vi "Lire fichiers config acqui.vi"(2 "error in (no error)":errorcluster caption="entrée d'erreur (pas d'erreur)") -> (0 "error out":errorcluster caption="sortie d'erreur")   [LabVIEW 2022 SP3]
uses:
  Variables globales/Variable glob Leybold.vi
  Variables globales/Variable glob Edwards.vi
  Variables globales/Variable glob Keller.vi
  Variables globales/Variables glob EUROTHERM.vi
  Variables globales/Variable globale compteurs.vi
  <vilib>/Utility/config.llb/NI_LVConfig.lvlib
panel:
  out "chemin complet":path
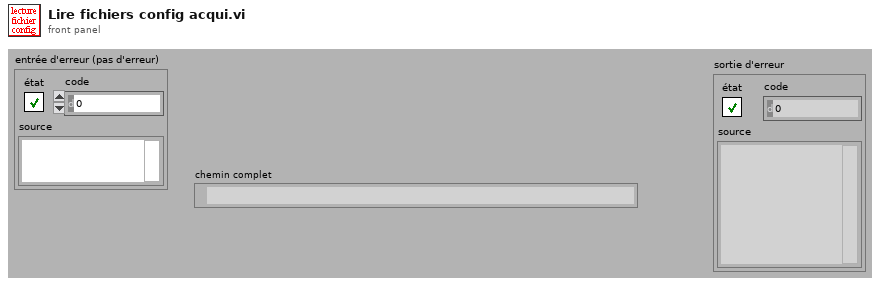
[diagram p1: front panel]
types:
  T1 = typedef "NI_LVConfig.lvlib/Config Data RefNum.ctl" = refnum<k1>
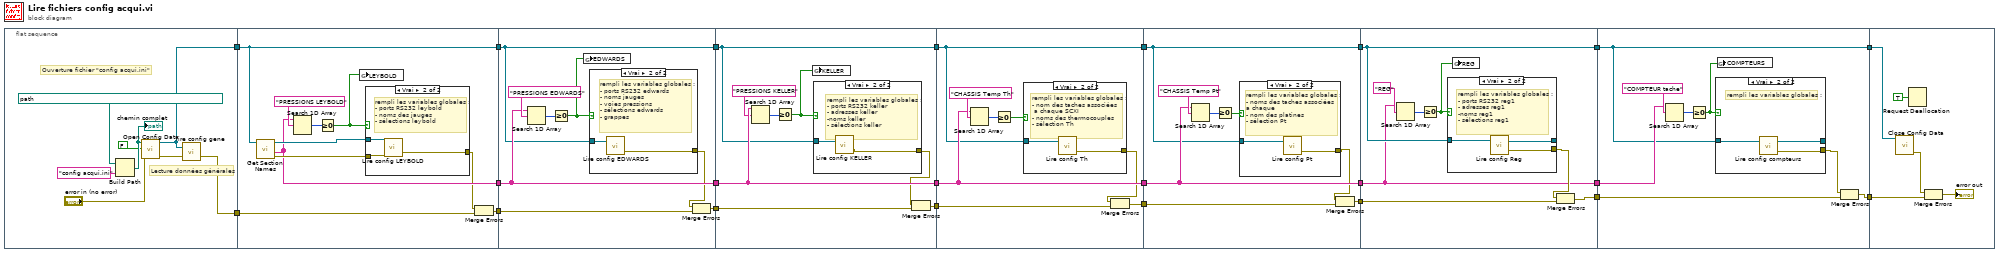
[diagram p0: block diagram]
diagram:
  n1 = flat-sequence {
    tunnel: [w26] -> w17
    tunnel: [w23] -> w16
    tunnel: w17 -> [w33]
    tunnel: [w35] -> w22
    tunnel: w16 -> [w34]
    tunnel: [w34] -> w15
    tunnel: [w31] -> w10
    tunnel: w22 -> [w49]
    tunnel: [w49] -> w21
    tunnel: w15 -> [w48]
    tunnel: [w48] -> w14
    tunnel: w10 -> [w47]
    tunnel: [w45] -> w9
    tunnel: w21 -> [w61]
    tunnel: [w61] -> w20
    tunnel: w14 -> [w58]
    tunnel: [w58] -> w13
    tunnel: w9 -> [w57]
    tunnel: [w55] -> w8
    tunnel: w20 -> [w69]
    tunnel: [w69] -> w19
    tunnel: w13 -> [w68]
    tunnel: [w68] -> w12
    tunnel: w8 -> [w67]
    tunnel: [w65] -> w7
    tunnel: w19 -> [w79]
    tunnel: [w79] -> w18
    tunnel: w12 -> [w78]
    tunnel: [w78] -> w11
    tunnel: w7 -> [w77]
    tunnel: [w75] -> w6
    tunnel: w18 -> [w85]
    tunnel: w11 -> [w89]
    tunnel: [w89] -> w5
    tunnel: w6 -> [w88]
    tunnel: [w87] -> w3
    tunnel: [w85] -> w1
    tunnel: w5 -> [w100]
    tunnel: [w100] -> w4
    tunnel: w3 -> [w98]
    tunnel: [w97] -> w2
    tunnel: w1 -> [w101]
    tunnel: w4 -> [w112]
    tunnel: w2 -> [w111]
    frame #0 {
      # "Lecture données générales"
      # "Ouverture fichier \"config acqui.ini\""
      n2 = Build Path(base path=path "C:/LABVIEW/PRES+TEMP+REG dernière version/Configurations", name or relative path="config acqui.ini" ("nom ou chemin relatif")) -> (appended path=w30:path)
      "chemin complet" <- w30
      n3 = call <vilib>:"Open Config Data.vi"("error in (no error)"="error in (no error)", "create file if necessary (T)"=FALSE ("create file if necessary? (T)"), "configuration file path"=w30) -> ("error out"=w27:errorcluster, "refnum"=w23:T1)  [unwired: 6 in, 1 out]
      n4 = call "lire config gene.vi"("error in"=w27, "refnum"=w23) -> ("error out"=w26:errorcluster)  [unwired: 1 out]
    }
    frame #1 {
      n5 = call <vilib>:"Get Section Names.vi"("refnum"=w34) -> ("error out"=w37:errorcluster, "section names"=w35:string[], "refnum out"=w38:T1)  [unwired: 8 in]
      n6 = Search 1D Array(1D array=w35, element="PRESSIONS LEYBOLD") -> (index of element=w39:i32)  [unwired: 1 in]
      n7 = Greater Or Equal To 0?(x=w39) -> (x >= 0?=w36:bool)
      n8 = global write "Variable glob Leybold.vi" "LEYBOLD"(w36) -> ()
      n9 = case shown="Vrai" w36 {
        tunnel: w38 -> [_ w44]
        tunnel: w37 -> [w41 w43]
        tunnel: [w41 w42] -> w32
        frame False {
          # "Pas de jauges\nLEYBOLD"
        }
        frame True {
          # "rempli les variables globales :\n- ports RS232 leybold\n- noms des jauges\n- sélections leybold"
          n10 = call "Lire config LEYBOLD.vi"("error in (no error)"=w43, "refnum"=w44) -> ("error out"=w42:errorcluster)  [unwired: 1 out]
        }
      }
      n11 = Merge Errors(w32, w33) -> (w31:errorcluster)
    }
    frame #2 {
      n12 = Search 1D Array(1D array=w49, element="PRESSIONS EDWARDS") -> (index of element=w51:i32)  [unwired: 1 in]
      n13 = Greater Or Equal To 0?(x=w51) -> (x >= 0?=w52:bool)
      n14 = global write "Variable glob Edwards.vi" "EDWARDS"(w52) -> ()
      n15 = case shown="Vrai" w52 {
        tunnel: w48 -> [_ w54]
        tunnel: [_ w53] -> w46
        frame False {
          # "Pas de jauges\nEDWARDS"
        }
        frame True {
          # "rempli les variables globales :\n- ports RS232 edwards\n- noms jauges\n- voies pressions\n- sélections edwards\n- grappes"
          n16 = call "Lire config EDWARDS.vi"("refnum"=w54) -> ("error out"=w53:errorcluster)  [unwired: 1 in, 1 out]
        }
      }
      n17 = Merge Errors(w46, w47) -> (w45:errorcluster)
    }
    frame #3 {
      n18 = Search 1D Array(1D array=w61, element="PRESSIONS KELLER") -> (index of element=w62:i32)  [unwired: 1 in]
      n19 = Greater Or Equal To 0?(x=w62) -> (x >= 0?=w59:bool)
      n20 = global write "Variable glob Keller.vi" "KELLER"(w59) -> ()
      n21 = case shown="Vrai" w59 {
        tunnel: w58 -> [_ w64]
        tunnel: [_ w63] -> w56
        frame False {
          # "Pas de jauges\nKELLER"
        }
        frame True {
          # "rempli les variables globales :\n- ports RS232 keller\n- adresses keller\n-noms keller\n- sélections keller"
          n22 = call "Lire config KELLER.vi"("refnum"=w64) -> ("error out"=w63:errorcluster)  [unwired: 1 in, 1 out]
        }
      }
      n23 = Merge Errors(w56, w57) -> (w55:errorcluster)
    }
    frame #4 {
      n24 = Search 1D Array(1D array=w69, element="CHASSIS Temp Th") -> (index of element=w72:i32)  [unwired: 1 in]
      n25 = Greater Or Equal To 0?(x=w72) -> (x >= 0?=w70:bool)
      n26 = case shown="Vrai" w70 {
        tunnel: w68 -> [_ w74]
        tunnel: [_ w73] -> w66
        frame False {
        }
        frame True {
          # "rempli les variables globales :\n- nom des taches associées\n a chaque SCXI\n- noms des thermocouples\n- sélection Th"
          n27 = call "Lire config Th.vi"("refnum"=w74) -> ("error out"=w73:errorcluster)  [unwired: 1 in, 1 out]
        }
      }
      n28 = Merge Errors(w66, w67) -> (w65:errorcluster)
    }
    frame #5 {
      n29 = Search 1D Array(1D array=w79, element="CHASSIS Temp Pt" ("section")) -> (index of element=w82:i32)  [unwired: 1 in]
      n30 = Greater Or Equal To 0?(x=w82) -> (x >= 0?=w81:bool)
      n31 = case shown="Vrai" w81 {
        tunnel: w78 -> [_ w84]
        tunnel: [_ w83] -> w76
        frame False {
        }
        frame True {
          # "rempli les variables globales :\n- noms des taches associées \na chaque \n- nom des platines\n- sélection Pt"
          n32 = call "Lire config Pt.vi"("refnum"=w84) -> ("error out"=w83:errorcluster)  [unwired: 1 in, 1 out]
        }
      }
      n33 = Merge Errors(w76, w77) -> (w75:errorcluster)
    }
    frame #6 {
      n34 = Search 1D Array(1D array=w85, element="REG" ("section")) -> (index of element=w91:i32)  [unwired: 1 in]
      n35 = Greater Or Equal To 0?(x=w91) -> (x >= 0?=w90:bool)
      n36 = case shown="Vrai" w90 {
        tunnel: w89 -> [w93 w96]
        tunnel: [_ w95] -> w86
        tunnel: [w93 w94] -> _
        frame False {
        }
        frame True {
          # "rempli les variables globales :\n- ports RS232 reg1\n- adresses reg1\n-noms reg1\n- sélections reg1"
          n37 = call "Lire config Reg.vi"("refnum"=w96) -> ("error out"=w95:errorcluster, "refnum out"=w94:T1)  [unwired: 1 in]
        }
      }
      n38 = global write "Variables glob EUROTHERM.vi" "REG"(w90) -> ()
      n39 = Merge Errors(w86, w88) -> (w87:errorcluster)
    }
    frame #7 {
      n40 = Search 1D Array(1D array=w101, element="COMPTEUR tache" ("section")) -> (index of element=w103:i32)  [unwired: 1 in]
      n41 = Greater Or Equal To 0?(x=w103) -> (x >= 0?=w99:bool)
      n42 = case shown="Vrai" w99 {
        tunnel: w100 -> [w105 w108]
        tunnel: [_ w107] -> w104
        tunnel: [w105 w106] -> _
        frame False {
        }
        frame True {
          # "rempli les variables globales :"
          n43 = call "Lire config compteurs.vi"("refnum"=w108) -> ("error out"=w107:errorcluster, "refnum out"=w106:T1)  [unwired: 1 in]
        }
      }
      n44 = global write "Variable globale compteurs.vi" "COMPTEURS"(w99) -> ()
      n45 = Merge Errors(w104, w98) -> (w97:errorcluster)
    }
    frame #8 {
      n46 = call <vilib>:"Close Config Data.vi"("refnum"=w112) -> ("error out"=w110:errorcluster)  [unwired: 9 in, 1 out]
      n47 = Request Deallocation(TRUE ("flag")) -> ()
      n48 = Merge Errors(w110, w111) -> (→"error out":errorcluster)
    }
  }
